vi "async convert file.vi"(4 "error queue":refnum<queue>, 6 "Message Completion Handler":refnum<class "Message Completion Handler.lvclass">, 10 "session data":refnum<data-value>, 11 "TDMS File":path) -> ()   [LabVIEW 2020, in "Nominal-TDMS-Upload.lvlib" / "Nominal-TDMS-Upload.lvclass"]
uses:
  Nominal-TDMS-Upload.lvclass
  <vilib>/FlexLogger/SDK/PluginSDK.lvlibp/PEFClasses/SDK/Message Completion Handler/Message Completion Handler.lvclass
  <vilib>/Nominal/Nominal IO Client/lv_src/Nominal Client/Nominal Client.lvclass
  <vilib>/Nominal/Nominal IO Client/lv_src/datasources/dataset/dataset.lvclass
  <vilib>/Nominal/Nominal IO Client/submodules/nominal-streaming-labview-ffi/lv_src/Stream/Stream.lvclass
  <vilib>/Nominal/Nominal IO Client/submodules/nominal-streaming-labview-ffi/lv_src/Channel/Channel.lvclass
  <vilib>/Utility/miscctls.llb/LVMapReplaceAction.ctl
  stream reference data.ctl
panel:
  in  "error in (no error)":errorcluster
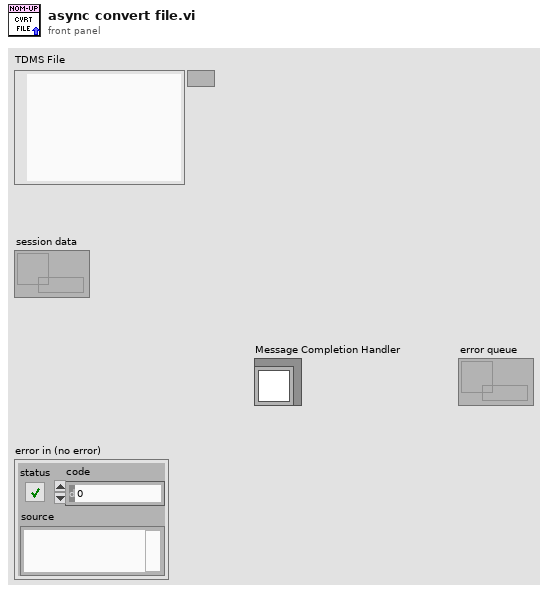
[diagram p1: front panel]
types:
  T1 = typedef "LVMapReplaceAction.ctl" = enum32{"Modify Entry only if found", "Add or Modify Entry", "Delete Entry"}
  T2 = typedef "Nominal-TDMS-Upload.lvlib/Nominal-TDMS-Upload.lvclass/stream reference data.ctl" = cluster{"Nominal Client":refnum<class "Nominal Client.lvclass">, "Dataset":refnum<class "dataset.lvclass">, "dataset stream":refnum<class "Stream.lvclass">, "Map":map{string, refnum<class "Channel.lvclass">}}
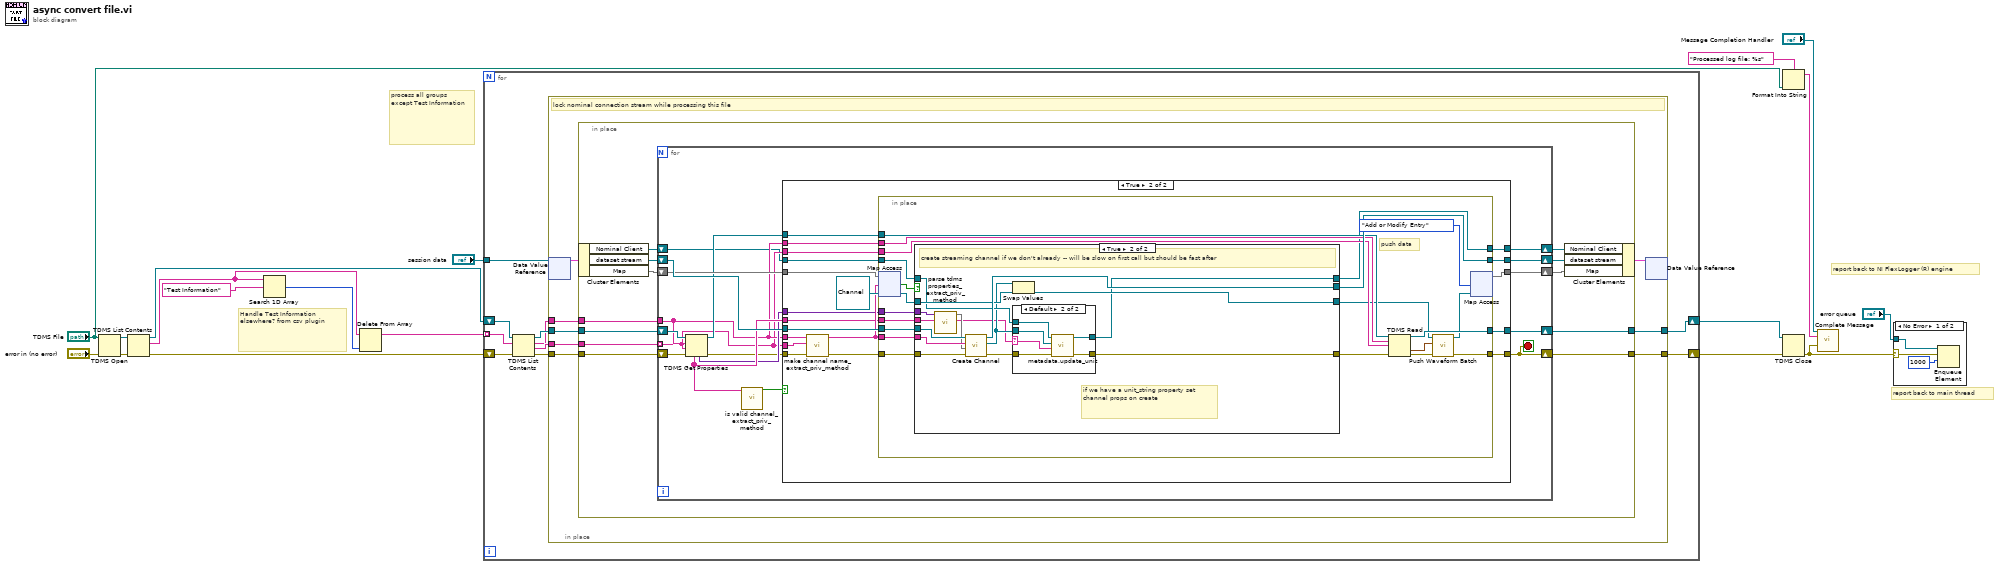
[diagram p0: block diagram]
diagram:
  # "report back to NI FlexLogger (R) engine"
  # "report back to main thread"
  # "process all groups except Test Information"
  # "Handle Test Information elsewhere? from csv plugin"
  n1 = TDMS Open(8:"error in (no error)", 11:"TDMS File") -> (0:w17:errorcluster, 3:w11:refnum<k34>)  [unwired: 5 in]
  n2 = TDMS List Contents(4:w17, 7:w11) -> (0:w13:errorcluster, 2:w15:string[], 3:w6:refnum<k34>)  [unwired: 1 in, 1 out]
  n3 = Search 1D Array(1D array=w15, element="Test Information" ("group name")) -> (index of element=w14:i32)  [unwired: 1 in]
  n4 = Delete From Array(array=w15, index=w14) -> (array with subset deleted=w5:string[])  [unwired: 1 in, 1 out]
  n5 = for {
    shift-right: [w24] -> w7
    shift-left: w13 -> [w28]
    shift-right: [w22] -> w1
    shift-left: w6 -> [w27]
    tunnel: w5 -> [w26] mode=indexing
    tunnel: "session data" -> [w23]
    n6 = TDMS List Contents(4:w28, 6:w26, 7:w27) -> (0:w25:errorcluster, 1:w21:string[], 2:w19:string, 3:w20:refnum<k34>)
    n7 = in-place {
      in-place-border: w25 -> [w36]
      in-place-border: [w35] -> w24
      in-place-border: w21 -> [w32]
      in-place-border: w20 -> [w31]
      in-place-border: [w30] -> w22
      in-place-border: w19 -> [w29]
      # "lock nominal connection stream while processing this file"
      n8 = in-place-dvr #1(w23) -> (w34:T2)  [unwired: 1 out]
      n9 = in-place {
        in-place-border: w36 -> [w48]
        in-place-border: [w47] -> w35
        in-place-border: w32 -> [w46]
        in-place-border: w31 -> [w41]
        in-place-border: [w40] -> w30
        in-place-border: w29 -> [w39]
        n10 = in-place-cluster #2(w34) -> ("Nominal Client"=w38:refnum<class "Nominal Client.lvclass">, "dataset stream"=w43:refnum<class "Stream.lvclass">, "Map"=w44:map{string, refnum<class "Channel.lvclass">})
        n11 = for {
          shift-right: [w60] -> w47
          shift-left: w48 -> [w55]
          tunnel: w46 -> [w51] mode=indexing
          shift-right: [w62] -> w42
          shift-left: w43 -> [w65]
          shift-right: [w64] -> w45
          shift-left: w44 -> [w63]
          shift-right: [w54] -> w40
          shift-left: w41 -> [w61]
          tunnel: w39 -> [w52]
          shift-right: [w49] -> w37
          shift-left: w38 -> [w50]
          stop <- w60 stop-if-true
          n12 = TDMS Get Properties(8:w55, 9:w51, 10:w52, 11:w61) -> (0:w56:errorcluster, 3:w53:refnum<k34>, 4:w57:variant[], 6:w58:string[])  [unwired: 2 in, 2 out]
          n13 = call "is valid channel_extract_priv_method.vi"("property names"=w58) -> ("Valid Channel"=w59:bool)  [unwired: 10 in]
          n14 = case shown="True" w59 {
            tunnel: w65 -> [w68 w89]
            tunnel: [w70 w88] -> w64
            tunnel: w63 -> [w70 w87]
            tunnel: [w68 w85] -> w62
            tunnel: [w69 w84] -> w60
            tunnel: w52 -> [_ w83]
            tunnel: w51 -> [_ w82]
            tunnel: w56 -> [w69 w80]
            tunnel: w58 -> [_ w78]
            tunnel: w57 -> [_ w77]
            tunnel: [w67 w76] -> w54
            tunnel: w53 -> [w67 w75]
            tunnel: w52 -> [_ w74]
            tunnel: w51 -> [_ w73]
            tunnel: w50 -> [w66 w72]
            tunnel: [w66 w71] -> w49
            frame False {
            }
            frame True {
              n15 = call "make channel name_extract_priv_method.vi"("error in (no error)"=w80, "channel name"=w82, "group name"=w83) -> ("error out"=w79:errorcluster, "qualified channel"=w81:string)  [unwired: 7 in]
              n16 = in-place {
                in-place-border: w79 -> [w110]
                in-place-border: [w94] -> w84
                in-place-border: w81 -> [w109]
                in-place-border: w89 -> [w108]
                in-place-border: [w107] -> w85
                in-place-border: w78 -> [w103]
                in-place-border: w77 -> [w102]
                in-place-border: w75 -> [w101]
                in-place-border: [w100] -> w76
                in-place-border: w74 -> [w99]
                in-place-border: w73 -> [w98]
                in-place-border: w72 -> [w91]
                in-place-border: [w90] -> w71
                # "push data"
                n17 = in-place-map #3(w87, w81, refnum<class "Channel.lvclass"> refnum ("channel")) -> (w104:refnum<class "Channel.lvclass">, w106:bool)
                n18 = case shown="True" w106 {
                  tunnel: w110 -> [w113 w129]
                  tunnel: [w113 w117] -> w97
                  tunnel: w109 -> [_ w128]
                  tunnel: w108 -> [w114 w127]
                  tunnel: [w114 w126] -> w107
                  tunnel: [w112 w125] -> w96
                  tunnel: w104 -> [w112 w124]
                  tunnel: w103 -> [_ w122]
                  tunnel: w102 -> [_ w121]
                  tunnel: w91 -> [w111 w120]
                  tunnel: [w111 w119] -> w90
                  frame False {
                    # "channel already exists"
                  }
                  frame True {
                    # "if we have a unit_string property set channel props on create"
                    # "create streaming channel if we don't already -- will be slow on first call but should be fast after"
                    n19 = call "parse tdms properties_extract_priv_method.vi"("property names"=w122, "property values"=w121) -> ("channel units"=w115:string, "nominal-compatible properties"=w123:map{string, string})  [unwired: 8 in]
                    n20 = call <vilib>:"Create Channel.vi"("error in (no error)"=w129, "Tags"=w123, "Channel Name"=w128, "Nominal Streaming in"=w127) -> ("error out"=w118:errorcluster, "Channel"=w116:refnum<class "Channel.lvclass">, "Nominal Streaming out"=w126:refnum<class "Stream.lvclass">)  [unwired: 5 in]
                    n21 = Swap Values(12:w116, 14:w124) -> (3:w125:refnum<class "Channel.lvclass">)  [unwired: 1 in, 1 out]
                    n22 = case shown="Default" w115 {
                      selector: w115 -> [_ w132]
                      tunnel: w120 -> [w131 w137]
                      tunnel: [w131 w136] -> w119
                      tunnel: w118 -> [w130 w135]
                      tunnel: [w130 w134] -> w117
                      tunnel: w116 -> [_ w133]
                      frame "" {
                      }
                      frame Default {
                        n23 = call <vilib>:"metadata.update_unit.vi"("error in"=w135, "Unit (empty to clear)"=w132, "Channel"=w133, "Nominal Client in"=w137) -> ("error out"=w134:errorcluster, "Nominal Client out"=w136:refnum<class "Nominal Client.lvclass">)  [unwired: 5 in, 1 out]
                      }
                    }
                  }
                }
                n24 = TDMS Read(0:w101, 5:w99, 7:w98, 11:w97) -> (4:w100:refnum<k34>, 10:w92:waveform(dbl), 15:w93:errorcluster)  [unwired: 4 in, 3 out]
                n25 = call <vilib>:"Push Waveform Batch.vi"("error in (no error)"=w93, "Waveform"=w92, "Channel in"=w96) -> ("error out"=w94:errorcluster, "Channel out"=w95:refnum<class "Channel.lvclass">)  [unwired: 7 in]
                n26 = in-place-map #3(w95, LVMapReplaceAction."Add or Modify Entry" ("action")) -> (w88:map{string, refnum<class "Channel.lvclass">})  [unwired: 2 out]
              }
            }
          }
        }
        n27 = in-place-cluster #2("Nominal Client"=w37, "dataset stream"=w42, "Map"=w45) -> (w33:T2)
      }
      n28 = in-place-dvr #1(w33) -> ()  [unwired: 2 out]
    }
  }
  n29 = Format Into String(format string="Processed log file: %s", "TDMS File") -> (resulting string=w9:string)  [unwired: 2 in, 1 out]
  n30 = TDMS Close(8:w7, 11:w1) -> (0:w2:errorcluster)  [unwired: 1 out]
  n31 = call-dynamic "Complete Message.vi"("MessageCompletionHandler in"="Message Completion Handler", "Reply Payload"=w9, "reply status"=w2) -> ()  [unwired: 11 in, 2 out]
  n32 = case shown="No Error" w2 {
    selector: w2 -> [w139 _]
    tunnel: "error queue" -> [w140 _]
    frame No Error {
      n33 = Enqueue Element(queue=w140, element=w139, timeout in ms (-1)=1000) -> ()  [unwired: 1 in, 3 out]
    }
    frame Error {
    }
  }
